vi "Panel.vi"(11 "ButtonControlEditorPanel in":refnum<class "NumericButtonEditorPanel.lvclass">) -> ()   [LabVIEW 2025, in "VolatusGUIControls.lvlib" / "NumericButtonEditorPanel.lvclass"]
uses:
  NumericButtonEditorPanel.lvclass
  NumericButtonEditorPanel.lvclass/NumericButtonEditorPanel.ctl
  C:/dev/volatus/mts-volatus-super/libs/volatus-gui-controls/VolatusGUIEditorCore/ElementEditorPanel/ElementEditorPanel.lvclass
  C:/dev/volatus/mts-volatus-super/libs/lv-oopanel/OOPanel/Panel/Panel.lvclass
  C:/dev/volatus/mts-volatus-super/libs/volatus-gui-controls/VolatusGUIControls/NumericButtonEditorPanel/NumericButtonEditorPanel.lvclass
  lv-oopanel/OOPanel/Panel/Basic UI State.ctl
  lv-oopanel/OOPanel/Panel/Panel.lvclass
  lv-oopanel/OOPanel/OOPanel.lvlib
  VolatusGUIControls.lvlib
  VolatusGUIEditorCore/ElementEditorPanel/ElementEditorPanel.lvclass
  lv-autocomplete/AutoComplete/AutoComplete/AutoComplete.lvclass
  31a50c44-4b6b-485d-bc13-bfcd23764fd1.vi
  VolatusGUIEditorCore/VolatusGUIEditorCore.lvlib
  03e8aef8-299f-4e90-a8ff-d58387ca9363.vi
panel:
  in  "Value":dbl
  in  "Top":i32
  in  "Left":i32
  in  "Height":u16
  in  "Width":u16
  in  "Label Text Color":u32(colorbox) caption="Color"
  in  "Text Color":u32(colorbox)
  in  "Label Visible":bool caption="Visible"
  in  "Label":string
  in  "Multi":bool
  in  "Channel":string
  in  "True Color":u32(colorbox)
  in  "False Color":u32(colorbox)
  in  "True Text":string
  in  "False Text":string
  # "Label"
  # "False"
  # "True"
  # "Text"
  # "BG"
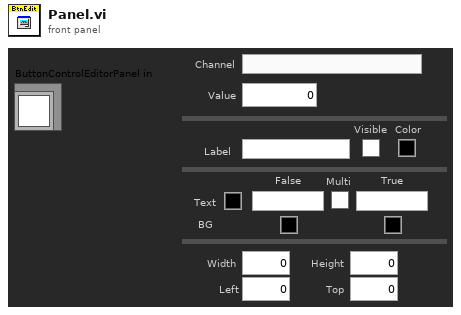
[diagram p1: front panel]
types:
  T1 = typedef "OOPanel.lvlib/Panel.lvclass/Basic UI State.ctl" = enum16{"Init", "Run", "Close"}
  T2 = typedef "VolatusGUIEditorCore.lvlib/ElementEditorPanel.lvclass/Incoming Events.ctl" = cluster{"Update Control":refnum<user-event>}
  T3 = typedef "OOPanel.lvlib/Panel.lvclass/Panel Events.ctl" = cluster{"Visbility":refnum<user-event>, "Close":refnum<user-event>}
  T4 = typedef "VolatusGUIControls.lvlib/NumericButtonEditorPanel.lvclass/Props.ctl" = cluster{"JSON":T5, "Label":T6, "Position":T7, "Width":u16, "Height":u16, "Boolean Colors":T8, "Boolean Text Props":T9}
  T5 = typedef "VolatusGUIControls.lvlib/NumericButtonEditorPanel.lvclass/JSON Props.ctl" = cluster{"Channel":string, "Value":dbl}
  T6 = typedef "VolatusGUIEditorCore.lvlib/Label Props.ctl" = cluster{"Text":string, "Text Color":u32, "Visible":bool}
  T7 = typedef "VolatusGUIEditorCore.lvlib/Position Props.ctl" = cluster{"Left":i32, "Top":i32}
  T8 = typedef "VolatusGUIEditorCore.lvlib/Boolean Color Props.ctl" = cluster{"False":u32, "True":u32}
  T9 = typedef "VolatusGUIEditorCore.lvlib/Boolean Text Props.ctl" = cluster{"Color":u32, "MultiString":bool, "False":string, "True":string, "Visible":bool}
  T10 = typedef "OOPanel.lvlib/Visibility State.ctl" = enum16{"Idle", "Closed", "Hidden", "Visible", "Subpanel", "Hidden Subpanel"}
  T11 = cluster{"Label":string, "Label Text Color":u32, "Label Visible":bool}
  T12 = cluster{"Text Color":u32, "Multi":bool, "False Text":string, "True Text":string, "Visible":bool}
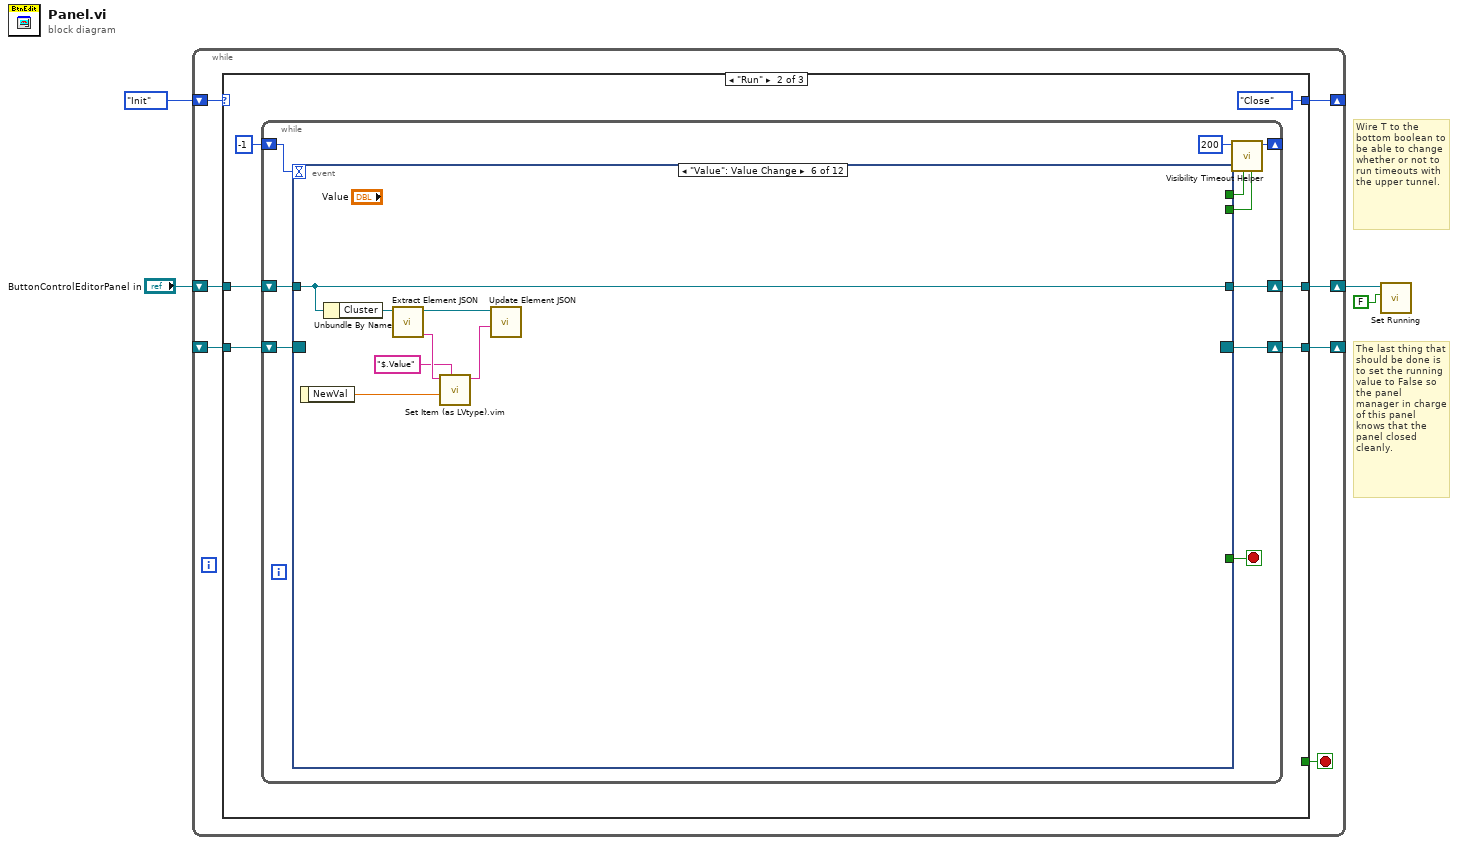
[diagram p0: block diagram]
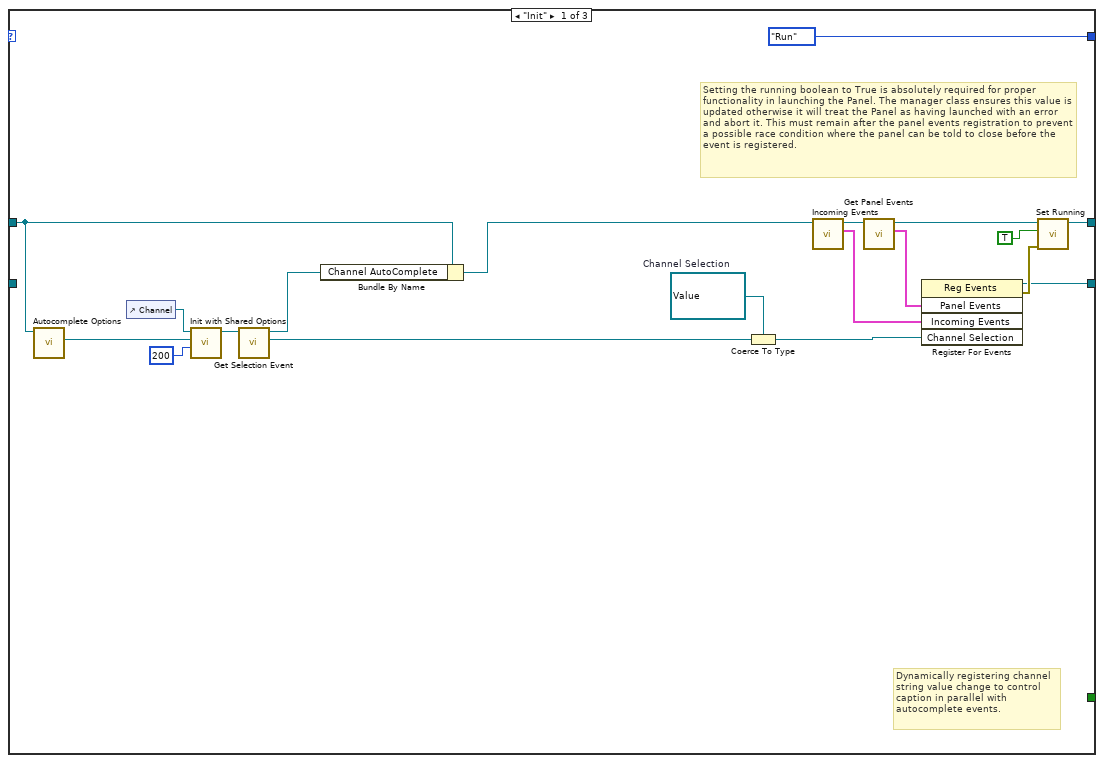
[diagram p2: hidden frame]
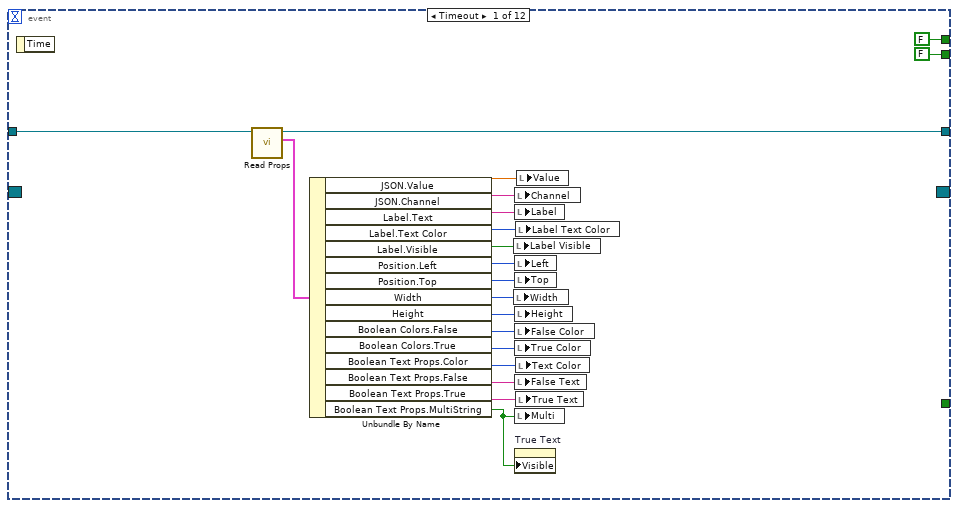
[diagram p3: hidden frame]
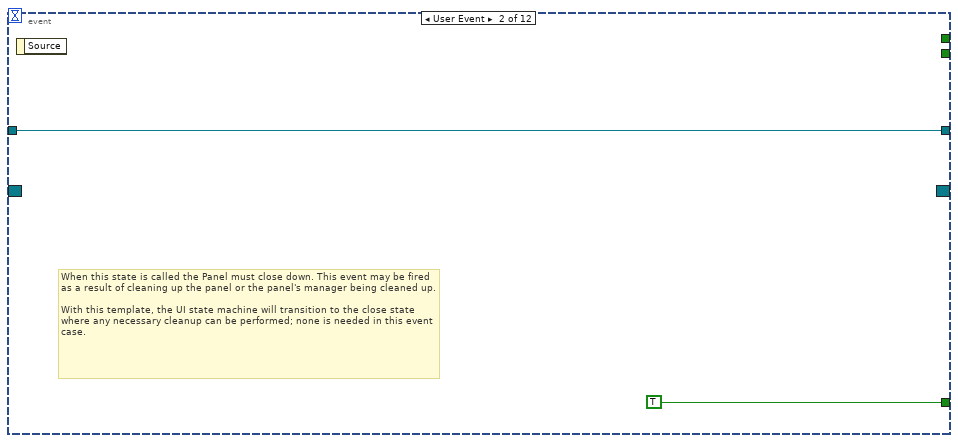
[diagram p4: hidden frame]
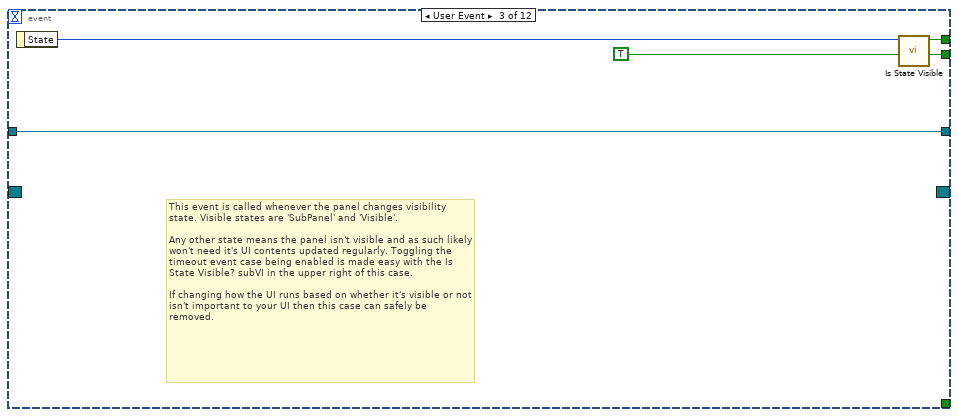
[diagram p5: hidden frame]
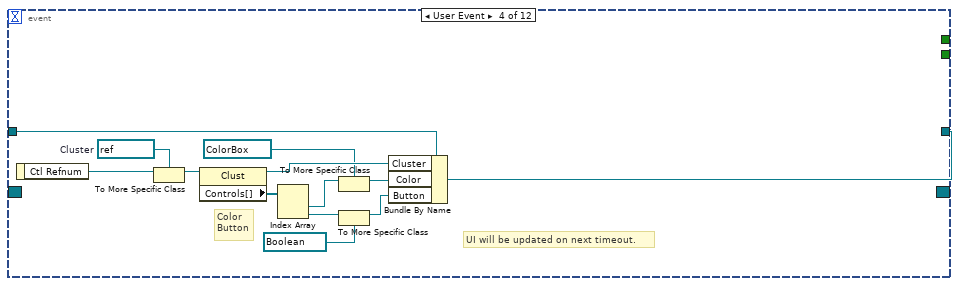
[diagram p6: hidden frame]
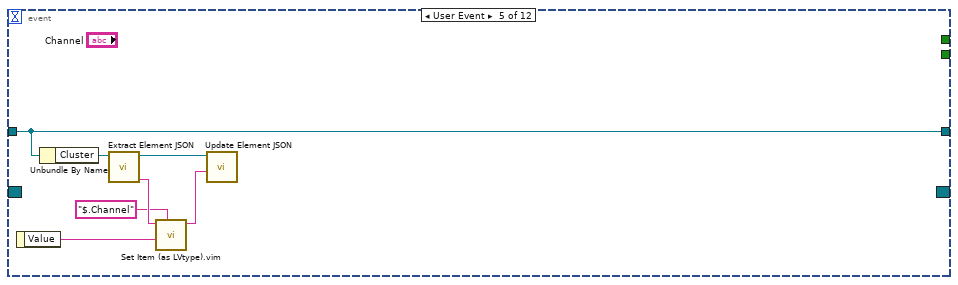
[diagram p7: hidden frame]
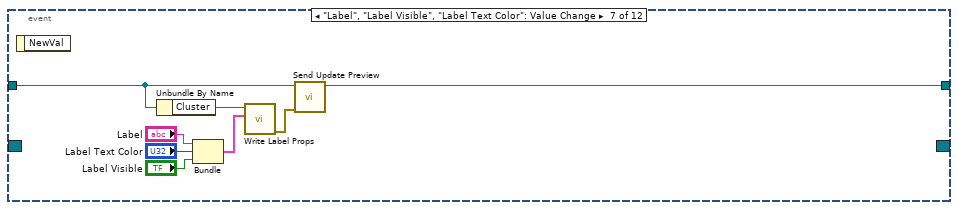
[diagram p8: hidden frame]
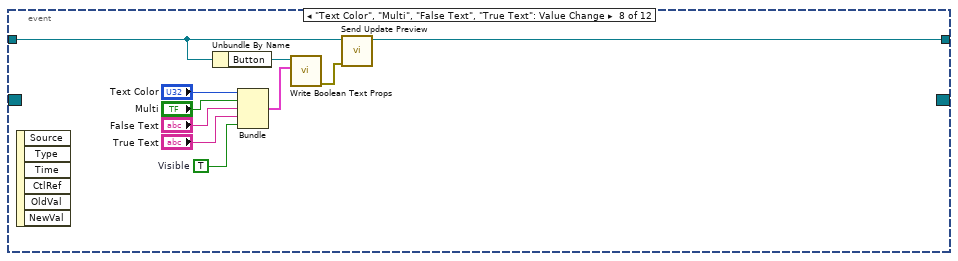
[diagram p9: hidden frame]
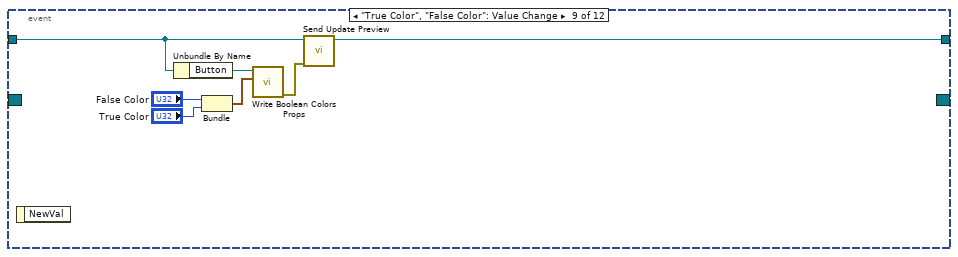
[diagram p10: hidden frame]
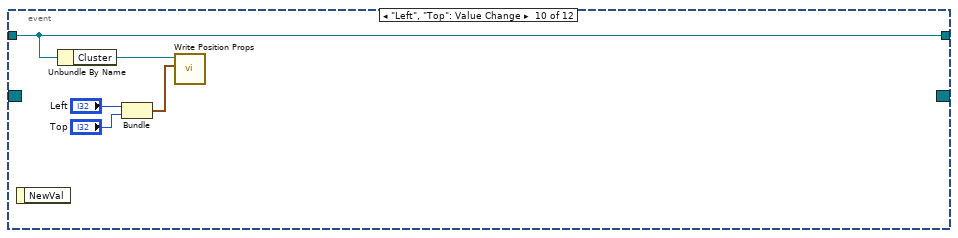
[diagram p11: hidden frame]
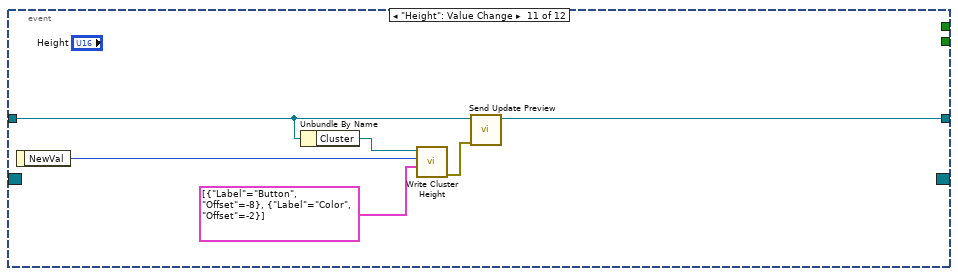
[diagram p12: hidden frame]
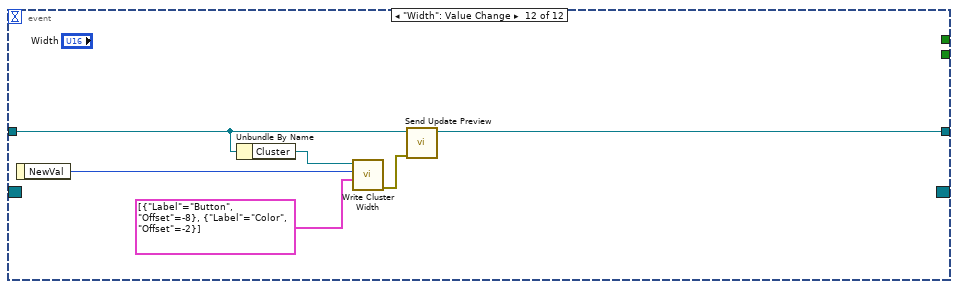
[diagram p13: hidden frame]
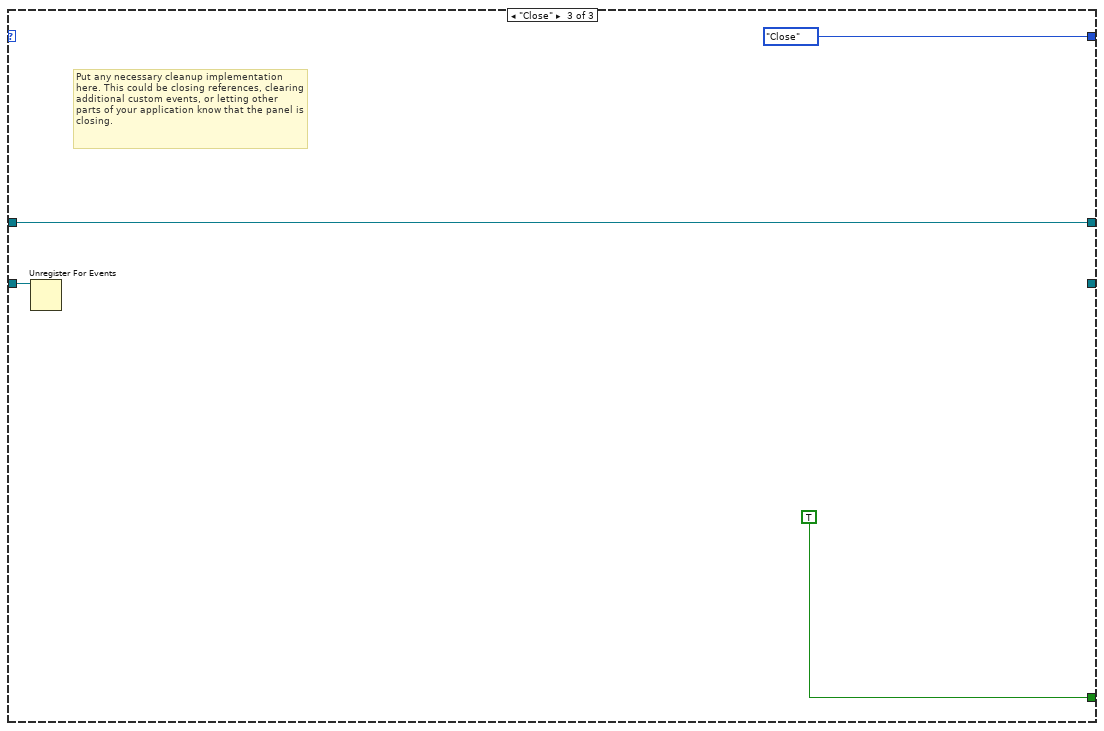
[diagram p14: hidden frame]
diagram:
  # "The last thing that should be done is to set the running value to False so the panel manager in charge of this panel knows that the panel closed cleanly."
  # "Wire T to the bottom boolean to be able to change whether or not to run timeouts with the upper tunnel."
  n1 = while {
    shift-right: [w10] -> _
    shift-left: _ -> [w11]
    shift-right: [w8] -> _
    shift-left: Basic_UI_State."Init" ("Basic UI State") -> [w9]
    shift-right: [w6] -> w4
    shift-left: "ButtonControlEditorPanel in" -> [w5]
    stop <- w7 stop-if-true
    n2 = case shown="\"Run\"" w9 {
      tunnel: w11 -> [_ w36 w143]
      tunnel: [w27 w34 _] -> w10
      tunnel: [Basic_UI_State."Run" ("Basic UI State") Basic_UI_State."Close" ("Basic UI State") Basic_UI_State."Close" ("Basic UI State")] -> w8
      tunnel: [_ _ TRUE] -> w7
      tunnel: [w26 w31 w142] -> w6
      tunnel: w5 -> [w23 w32 w142]
      frame "Init" {
        w12 = refnum<user-event> refnum  # Channel Selection
        # "Dynamically registering channel string value change to control caption in parallel with autocomplete events."
        # "Setting the running boolean to True is absolutely required for proper functionality in launching the Panel. The manager class ensures this value is updated otherwise it will treat the Panel as having launched with an error and abort it. This must remain after the panel events registration to prevent a possible race condition where the panel can be told to close before the event is registered."
        n3 = call "Autocomplete Options.vi"("ElementEditorPanel in"=w23) -> ("Autocomplete Options"=w14:refnum<class "Shared Options.lvclass">)  [unwired: 10 in]
        n4 = control-ref of="Channel"() -> (w22:refnum<vi>)
        n5 = call "Init with Shared Options.vi"("Height (200)"=i16 200, "Shared Options"=w14, "Str Refnum"=w22) -> ("AutoComplete out"=w21:refnum<class "AutoComplete.lvclass">)  [unwired: 7 in, 1 out]
        n6 = call "Get Selection Event.vi"("AutoComplete in"=w21) -> ("Selection Event"=w20:refnum<user-event>, "AutoComplete"=w18:refnum<class "AutoComplete.lvclass">)  [unwired: 9 in]
        n7 = Bundle By Name(cluster=w23, "Channel AutoComplete"=w18) -> (w16:refnum<class "NumericButtonEditorPanel.lvclass">)
        n8 = Coerce To Type(0:w20, 1:w12) -> (2:w13:refnum<user-event>)
        n9 = call "Incoming Events.vi"("ElementEditorPanel in"=w16) -> ("Incoming Events"=w17:T2, "ElementEditorPanel out"=w15:refnum<class "NumericButtonEditorPanel.lvclass">)  [unwired: 9 in]
        n10 = call "Get Panel Events.vi"("Panel in"=w15) -> ("Panel Events"=w24:T3, "Panel out"=w25:refnum<class "NumericButtonEditorPanel.lvclass">)  [unwired: 8 in, 1 out]
        n11 = register-events(w24, w17, w13) -> (reference out=w27:refnum<event-registration>, error out=w29:errorcluster)  [unwired: 2 in]
        n12 = call "Set Running.vi"("error in (no error)"=w29, "Running"=TRUE, "Panel in"=w25) -> ("Panel out"=w26:refnum<class "NumericButtonEditorPanel.lvclass">)  [unwired: 7 in, 1 out]
      }
      frame "Run" {
        n13 = while {
          shift-right: [w42] -> w34
          shift-left: w36 -> [w43]
          shift-right: [w45] -> _
          shift-left: -1 ("Timeout") -> [w44]
          shift-right: [w37] -> w31
          shift-left: w32 -> [w38]
          stop <- w39 stop-if-true
          n14 = event shown="[5] \"Value\": Value Change" {
            selector: w43 -> [_ _ _ _ _ _ _ _ _ _ _ _]
            dyn-events: [_ _ _ _ _ _ _ _ _ _ _ _] -> w42
            timeout: w44 -> [_ _ _ _ _ _ _ _ _ _ _ _]
            tunnel: [FALSE _ w71 _ _ _ _ _ _ _ _ _] -> w41
            tunnel: [FALSE _ TRUE _ _ _ _ _ _ _ _ _] -> w40
            tunnel: [_ TRUE _ _ _ _ _ _ _ _ _ _] -> w39
            tunnel: w38 -> [w62 w67 w69 w85 w92 w99 w107 w117 w124 w129 w132 w141]
            tunnel: [w61 w67 w69 w73 w92 w99 w106 w110 w123 w129 w130 w140] -> w37
            event Timeout {
              n15 = event-data() -> ()  [unwired: 1 in, 1 out]
              n16 = call "Read Props.vi"("ButtonControlEditorPanel in"=w62) -> ("Props"=w64:T4, "ButtonControlEditorPanel out"=w61:refnum<class "NumericButtonEditorPanel.lvclass">)  [unwired: 8 in, 1 out]
              n17 = Unbundle By Name(w64) -> ("JSON.Value"=w47:dbl, "JSON.Channel"=w63:string, "Label.Text"=w60:string, "Label.Text Color"=w58:u32, "Label.Visible"=w57:bool, "Position.Left"=w56:i32, "Position.Top"=w55:i32, "Width"=w54:u16, "Height"=w53:u16, "Boolean Colors.False"=w52:u32, "Boolean Colors.True"=w51:u32, "Boolean Text Props.Color"=w50:u32, "Boolean Text Props.False"=w49:string, "Boolean Text Props.True"=w59:string, "Boolean Text Props.MultiString"=w48:bool)
              n18 = local write "Label Visible"(w57) -> ()
              n19 = local write "Width"(w54) -> ()
              n20 = local write "Channel"(w63) -> ()
              n21 = local write "Label"(w60) -> ()
              n22 = local write "Left"(w56) -> ()
              n23 = local write "Top"(w55) -> ()
              n24 = local write "Height"(w53) -> ()
              n25 = local write "False Color"(w52) -> ()
              n26 = local write "True Color"(w51) -> ()
              n27 = local write "False Text"(w49) -> ()
              n28 = local write "Multi"(w48) -> ()
              n29 = property on="True Text" class="Str"("Visible"=w48) -> ()  [unwired: 2 in, 2 out]
              n30 = local write "Label Text Color"(w58) -> ()
              n31 = local write "Text Color"(w50) -> ()
              n32 = local write "True Text"(w59) -> ()
              n33 = local write "Value"(w47) -> ()
            }
            event User Event {
              # "When this state is called the Panel must close down. This event may be fired as a result of cleaning up the panel or the panel's manager being cleaned up.\n\nWith this template, the UI state machine will transition to the close state where any necessary cleanup can be performed; none is needed in this event case."
              n34 = event-data() -> ()  [unwired: 1 in, 1 out]
            }
            event User Event {
              # "This event is called whenever the panel changes visibility state. Visible states are 'SubPanel' and 'Visible'.\n\nAny other state means the panel isn't visible and as such likely won't need it's UI contents updated regularly. Toggling the timeout event case being enabled is made easy with the Is State Visible? subVI in the upper right of this case.\n\nIf changing how the UI runs based on whether it's visible or not isn't important to your UI then this case can safely be removed."
              n35 = event-data() -> ("State"=w72:T10)  [unwired: 1 in]
              n36 = call "Is State Visible.vi"("Visibility"=w72) -> ("Visible"=w71:bool)  [unwired: 10 in]
            }
            event User Event {
              w82 = refnum<vi> refnum  # Cluster
              # "UI will be updated on next timeout."
              # "Color\nButton"
              n37 = event-data() -> ("Ctl Refnum"=w84:refnum<vi>)  [unwired: 1 in]
              n38 = To More Specific Class(target class=w82, reference=w84) -> (specific class reference=w83:refnum<vi>)  [unwired: 1 in, 1 out]
              n39 = property class="Clust"(reference=w83) -> (reference out=w78:refnum<vi>, "Controls[]"=w81:refnum<vi>[])  [unwired: 1 in, 1 out]
              n40 = Index Array(array=w81) -> (element #1=w75:refnum<vi>, element #2=w80:refnum<vi>)  [unwired: 2 in]
              n41 = To More Specific Class(target class=refnum<vi> refnum ("False Color"), reference=w75) -> (specific class reference=w76:refnum<vi>)  [unwired: 1 in, 1 out]
              n42 = To More Specific Class(target class=refnum<vi> refnum ("Button"), reference=w80) -> (specific class reference=w77:refnum<vi>)  [unwired: 1 in, 1 out]
              n43 = Bundle By Name(cluster=w85, "Cluster"=w78, "Color"=w76, "Button"=w77) -> (w73:refnum<class "NumericButtonEditorPanel.lvclass">)
            }
            event User Event {
              n44 = event-data() -> ("Value"=w89:string)  [unwired: 1 in]
              n45 = Unbundle By Name(w92) -> ("Cluster"=w91:refnum<vi>)
              n46 = call "Extract Element JSON.vi"("Ctl Refnum in"=w91) -> ("JSON"=w90:string, "Ctl Refnum"=w87:refnum<vi>)  [unwired: 7 in, 2 out]
              n47 = call "Set Item (as LVtype).vim"("$Path or Item Name"="$.Channel", "Anything"=w89, "JSON"=w90) -> ("<JSON>"=w86:string)  [unwired: 5 in, 2 out]
              n48 = call "Update Element JSON.vi"("JSON"=w86, "Ctl Refnum in"=w87) -> ()  [unwired: 8 in, 2 out]
            }
            event "Value": Value Change {
              n49 = event-data() -> ("NewVal"=w96:dbl)  [unwired: 1 in]
              n50 = Unbundle By Name(w99) -> ("Cluster"=w98:refnum<vi>)
              n51 = call "Extract Element JSON.vi"("Ctl Refnum in"=w98) -> ("JSON"=w97:string, "Ctl Refnum"=w94:refnum<vi>)  [unwired: 7 in, 2 out]
              n52 = call "Set Item (as LVtype).vim"("$Path or Item Name"="$.Value", "Anything"=w96, "JSON"=w97) -> ("<JSON>"=w93:string)  [unwired: 5 in, 2 out]
              n53 = call "Update Element JSON.vi"("JSON"=w93, "Ctl Refnum in"=w94) -> ()  [unwired: 8 in, 2 out]
            }
            event "Label", "Label Visible", "Label Text Color": Value Change {
              n54 = event-data() -> ()  [unwired: 1 in, 1 out]
              n55 = Unbundle By Name(w107) -> ("Cluster"=w105:refnum<vi>)
              n56 = Bundle("Label"="Label", "Label Text Color"="Label Text Color", "Label Visible"="Label Visible") -> (w100:T11)  [unwired: 1 in]
              n57 = call "Write Label Props.vi"("Label Props"=w100, "Ctl Refnum in"=w105) -> ("error out"=w104:errorcluster)  [unwired: 8 in, 1 out]
              n58 = call "Send Update Preview.vi"("error in (no error)"=w104, "ElementEditorPanel in"=w107) -> ("ElementEditorPanel out"=w106:refnum<class "NumericButtonEditorPanel.lvclass">)  [unwired: 8 in, 1 out]
            }
            event "Text Color", "Multi", "False Text", "True Text": Value Change {
              w108 = TRUE  # Visible
              n59 = event-data() -> ()  [unwired: 1 in, 6 out]
              n60 = Unbundle By Name(w117) -> ("Button"=w112:refnum<vi>)
              n61 = Bundle("Text Color"="Text Color", "Multi"="Multi", "False Text"="False Text", "True Text"="True Text", "Visible"=w108) -> (w111:T12)  [unwired: 1 in]
              n62 = call "Write Boolean Text Props.vi"("Boolean Text Props"=w111, "Control In"=w112) -> ("error out"=w109:errorcluster)  [unwired: 8 in, 1 out]
              n63 = call "Send Update Preview.vi"("error in (no error)"=w109, "ElementEditorPanel in"=w117) -> ("ElementEditorPanel out"=w110:refnum<class "NumericButtonEditorPanel.lvclass">)  [unwired: 8 in, 1 out]
            }
            event "True Color", "False Color": Value Change {
              n64 = event-data() -> ()  [unwired: 1 in, 1 out]
              n65 = Unbundle By Name(w124) -> ("Button"=w122:refnum<vi>)
              n66 = Bundle("False Color"="False Color", "True Color"="True Color") -> (w119:cluster{"False Color":u32, "True Color":u32})  [unwired: 1 in]
              n67 = call "Write Boolean Colors Props.vi"("Boolean Colors Props"=w119, "Control in"=w122) -> ("error out"=w118:errorcluster)  [unwired: 8 in, 1 out]
              n68 = call "Send Update Preview.vi"("error in (no error)"=w118, "ElementEditorPanel in"=w124) -> ("ElementEditorPanel out"=w123:refnum<class "NumericButtonEditorPanel.lvclass">)  [unwired: 8 in, 1 out]
            }
            event "Left", "Top": Value Change {
              n69 = event-data() -> ()  [unwired: 1 in, 1 out]
              n70 = Unbundle By Name(w129) -> ("Cluster"=w128:refnum<vi>)
              n71 = Bundle("Left"="Left", "Top"="Top") -> (w125:cluster{"Left":i32, "Top":i32})  [unwired: 1 in]
              n72 = call "Write Position Props.vi"("Position Props"=w125, "Ctl Refnum in"=w128) -> ()  [unwired: 8 in, 2 out]
            }
            event "Height": Value Change {
              n73 = event-data() -> ("NewVal"=w131:u16)  [unwired: 1 in]
              n74 = Unbundle By Name(w132) -> ("Cluster"=w135:refnum<vi>)
              n75 = call "Write Cluster Height.vi"("Nested Offsets (None)"=cluster{"Label":string, "Offset":i32}[] [{"Label"="Button", "Offset"=-8}, {"Label"="Color", "Offset"=-2}], "Height"=w131, "Cluster in"=w135) -> ("error out"=w133:errorcluster)  [unwired: 7 in, 1 out]
              n76 = call "Send Update Preview.vi"("error in (no error)"=w133, "ElementEditorPanel in"=w132) -> ("ElementEditorPanel out"=w130:refnum<class "NumericButtonEditorPanel.lvclass">)  [unwired: 8 in, 1 out]
            }
            event "Width": Value Change {
              n77 = event-data() -> ("NewVal"=w138:u16)  [unwired: 1 in]
              n78 = Unbundle By Name(w141) -> ("Cluster"=w139:refnum<vi>)
              n79 = call "Write Cluster Width.vi"("Nested Offsets (None)"=cluster{"Label":string, "Offset":i32}[] [{"Label"="Button", "Offset"=-8}, {"Label"="Color", "Offset"=-2}], "Width"=w138, "Cluster in"=w139) -> ("error out"=w136:errorcluster)  [unwired: 7 in, 1 out]
              n80 = call "Send Update Preview.vi"("error in (no error)"=w136, "ElementEditorPanel in"=w141) -> ("ElementEditorPanel out"=w140:refnum<class "NumericButtonEditorPanel.lvclass">)  [unwired: 8 in, 1 out]
            }
          }
          n81 = call "Visibility Timeout Helper.vi"("Update?"=w40, "Use Timeout?"=w41, "Visible Timeout mS"=200) -> ("Timeout"=w45:i32)  [unwired: 8 in]
        }
      }
      frame "Close" {
        # "Put any necessary cleanup implementation here. This could be closing references, clearing additional custom events, or letting other parts of your application know that the panel is closing."
        n82 = Unregister For Events(event registration refnum=w143) -> ()  [unwired: 1 in, 1 out]
      }
    }
  }
  n83 = call "Set Running.vi"("Running"=FALSE, "Panel in"=w4) -> ()  [unwired: 8 in, 2 out]
